vi "RFH-read-general.vi"(7 "file path (dialog if empty)":path, 8 "error in":errorcluster, 11 "sim":bool) -> (0 "error out":errorcluster, 2 "Common Format":T1)   [LabVIEW 2020, in "RFH-Reflection_File_Handler.lvlib"]
doc: "Reads a measurement or simulation file (dialog if the path is empty) into a Common Format cluster; sim marks a simulation file."
uses:
  RFH-Reflection_File_Handler.lvlib
  RFH-common_data_format.ctl
  RFH-libreVNA_data_format.ctl
  <vilib>/Analysis/NI_AALPro.lvlib
panel:
  out "size(s)":i32
  out "real 2":dbl[](graph)
  out "imag 2":dbl[](graph)
  out "mag":dbl[](graph)
  out "phase":dbl[](graph)
  out "imag":dbl[](graph)
  out "real":dbl[](graph)
  out "freq":dbl[](graph)
  out "Array 2":string[](array[string])
  out "string array 3":string[](array[string])
  out "string array 2":string[][](array[string])
  out "string array":string[](array[string])
  out "after substring":string
  out "text":string
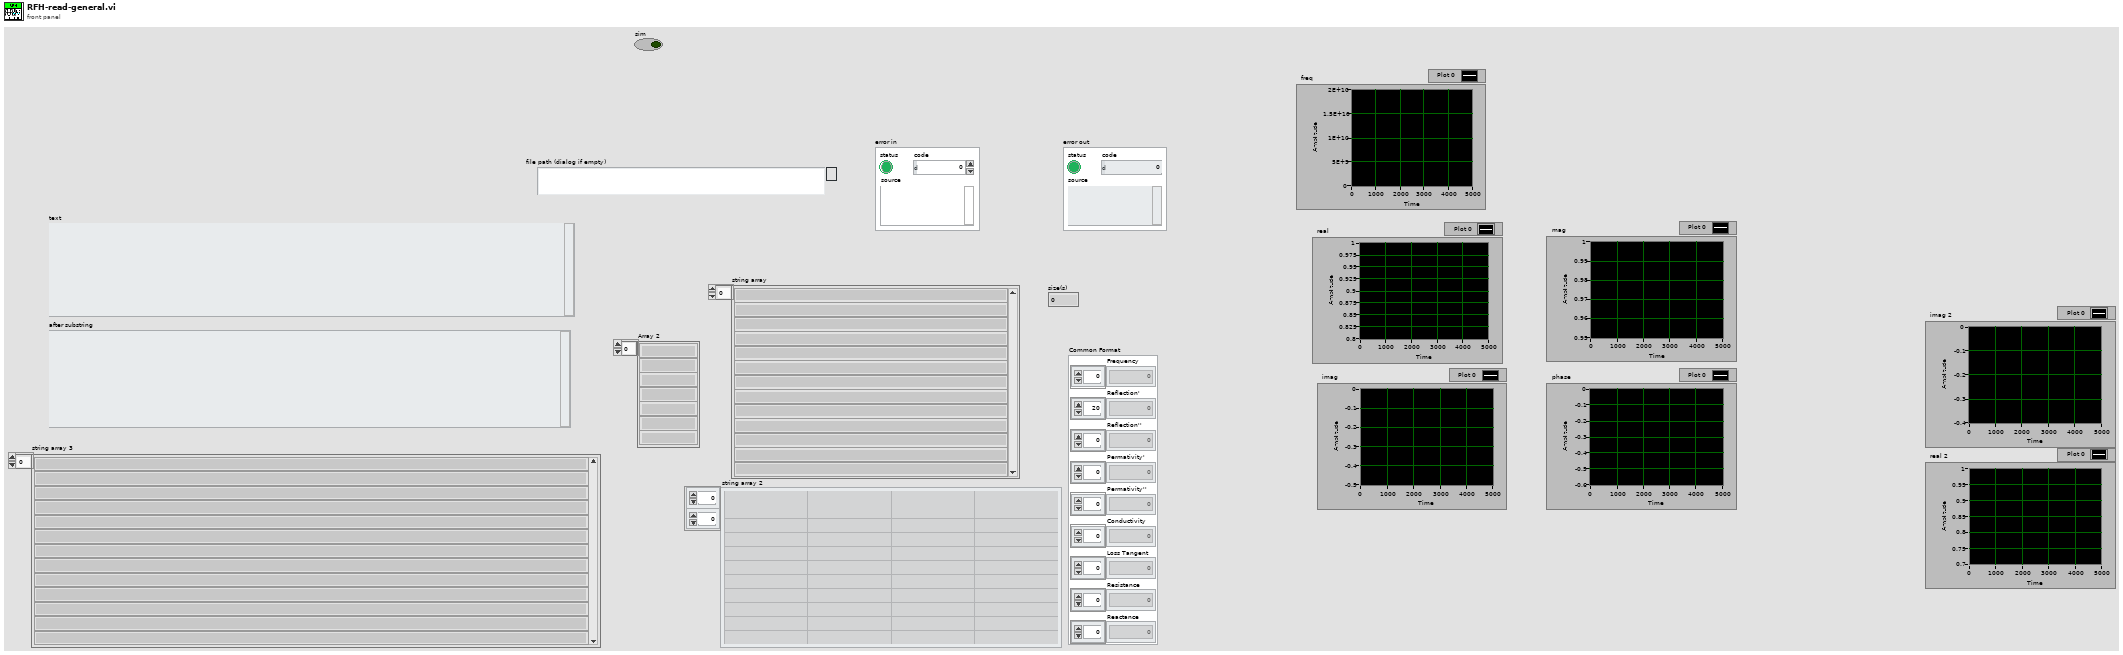
[diagram p1: front panel]
types:
  T1 = typedef "RFH-Reflection_File_Handler.lvlib/RFH-common_data_format.ctl" = cluster{"Frequency":dbl[], "Reflection'":dbl[], "Reflection''":dbl[], "Permativity'":dbl[], "Permativity''":dbl[], "Conductivity":dbl[], "Loss Tangent":dbl[], "Resistance":dbl[], "Reactance":dbl[]}
  T2 = typedef "RFH-Reflection_File_Handler.lvlib/RFH-libreVNA_data_format.ctl" = cluster{"Frequency":dbl[], "S11_Real":dbl[], "S11_Imag":dbl[], "S21_Real":dbl[], "S21_Imag":dbl[], "S12_Real":dbl[], "S12_Imag":dbl[], "S22_Real":dbl[], "S22_Imag":dbl[]}
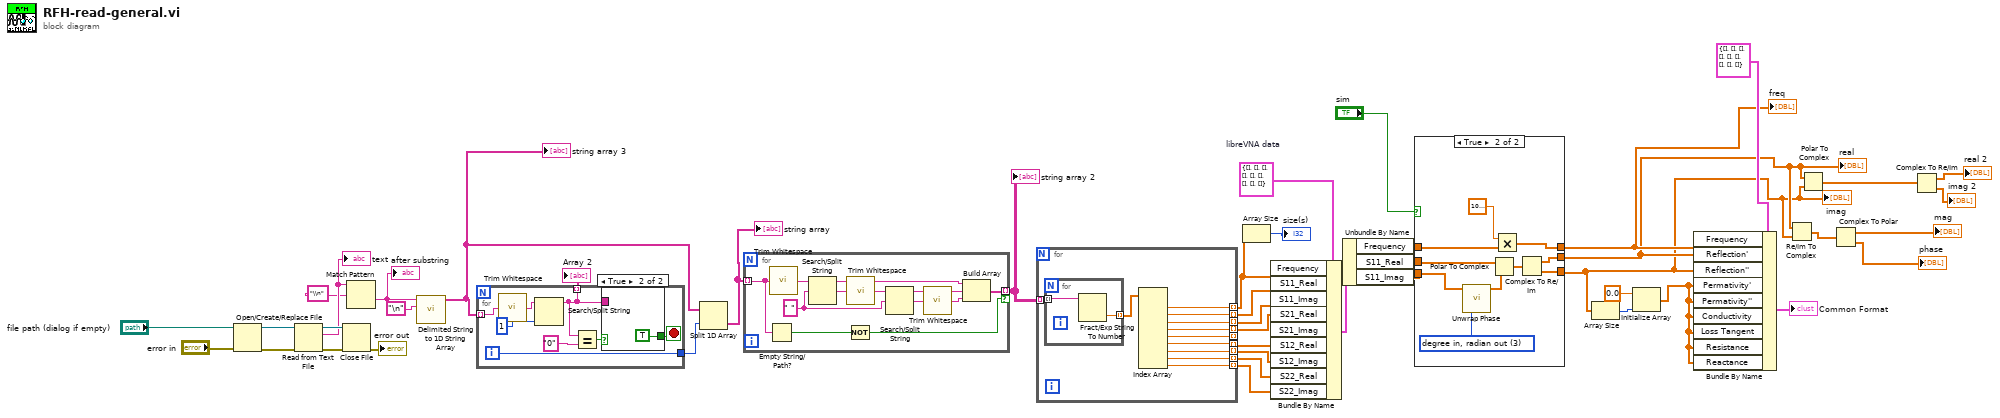
[diagram p0: block diagram]
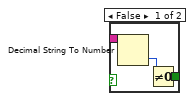
[diagram p3: hidden frame]
diagram:
  w29 = T2 {"Frequency"=[], "S11_Real"=[], "S11_Imag"=[], "S21_Real"=[], "S21_Imag"=[], "S12_Real"=[], "S12_Imag"=[], "S22_Real"=[], "S22_Imag"=[]}  # libreVNA data
  n1 = Open/Create/Replace File(file path (use dialog)="file path (dialog if empty)", error in="error in") -> (refnum out=w46:refnum<file>, error out=w43:errorcluster)  [unwired: 4 in, 1 out]
  n2 = Read from Text File(file (use dialog)=w46, error in=w43) -> (refnum out=w45:refnum<file>, text=w41:string, error out=w44:errorcluster)  [unwired: 2 in, 1 out]
  "text" <- w41
  n3 = Close File(refnum=w45, error in=w44) -> (error out=→"error out":errorcluster)  [unwired: 1 out]
  n4 = Match Pattern(string=w41, regular expression="\\n" ("search string/char (-)")) -> (after substring=w38:string)  [unwired: 1 in, 3 out]
  "after substring" <- w38
  n5 = call <vilib>:"Delimited String to 1D String Array.vi"("delimiter"="\n", "delimited string"=w38) -> ("string array"=w20:string[])  [unwired: 9 in]
  "string array 3" <- w20
  n6 = for {
    tunnel: w20 -> [w52] mode=indexing
    tunnel: [w54] -> w18
    tunnel: [w49] -> w17 mode=indexing
    i -> [w54]
    stop <- w50 stop-if-true
    n7 = call <vilib>:"Trim Whitespace.vi"("string"=w52) -> ("trimmed string"=w51:string)  [unwired: 1 in]
    n8 = Search/Split String(string=w51, offset (0)=1) -> (substring before match=w49:string)  [unwired: 1 in, 2 out]
    n9 = Equal?(x=w49, y="0") -> (x = y?=w47:bool)
    n10 = case shown="True" w47 {
      tunnel: [w56 TRUE] -> w50
      tunnel: w49 -> [w55 _]
      frame False {
        n11 = Decimal String To Number(string=w55) -> (number=w57:i32)  [unwired: 2 in, 1 out]
        n12 = Not Equal To 0?(x=w57) -> (x != 0?=w56:bool)
      }
      frame True {
      }
    }
  }
  "Array 2" <- w17
  n13 = Split 1D Array(array=w20, index=w18) -> (second subarray=w19:string[])  [unwired: 1 out]
  "string array" <- w19
  n14 = for {
    tunnel: w19 -> [w69] mode=indexing
    tunnel: [w59] -> w13 mode=indexing if=w68
    w64 = " " ("search string/char (-)")
    n15 = Empty String/Path?(string/path=w69) -> (empty?=w70:bool)
    n16 = call <vilib>:"Trim Whitespace.vi"("string"=w69) -> ("trimmed string"=w63:string)  [unwired: 1 in]
    n17 = Search/Split String(string=w63, search string/char (-)=w64) -> (substring before match=w62:string, match + rest of string=w66:string)  [unwired: 1 in, 1 out]
    n18 = Not(x=w70) -> (.not. x?=w68:bool)
    n19 = call <vilib>:"Trim Whitespace.vi"("string"=w66) -> ("trimmed string"=w67:string)  [unwired: 1 in]
    n20 = Search/Split String(string=w67, search string/char (-)=w64) -> (substring before match=w61:string, match + rest of string=w65:string)  [unwired: 1 in, 1 out]
    n21 = call <vilib>:"Trim Whitespace.vi"("string"=w65) -> ("trimmed string"=w60:string)  [unwired: 1 in]
    n22 = Build Array(w62, w61, w60) -> (w59:string[])
  }
  "string array 2" <- w13
  n23 = for {
    tunnel: w13 -> [w81] mode=indexing
    tunnel: [w79] -> w9 mode=indexing
    tunnel: [w78] -> w37 mode=indexing
    tunnel: [w77] -> w36 mode=indexing
    tunnel: [w76] -> w35 mode=indexing
    tunnel: [w75] -> w34 mode=indexing
    tunnel: [w74] -> w33 mode=indexing
    tunnel: [w73] -> w32 mode=indexing
    tunnel: [w72] -> w31 mode=indexing
    tunnel: [w71] -> w30 mode=indexing
    n24 = for {
      tunnel: w81 -> [w83] mode=indexing
      tunnel: [w82] -> w80 mode=indexing
      n25 = Fract/Exp String To Number(string=w83) -> (number=w82:dbl)  [unwired: 3 in, 1 out]
    }
    n26 = Index Array(array=w80) -> (element #1=w79:dbl, element #2=w78:dbl, element #3=w77:dbl, element #4=w76:dbl, element #5=w75:dbl, element #6=w74:dbl, element #7=w73:dbl, element #8=w72:dbl, element #9=w71:dbl)  [unwired: 9 in]
  }
  n27 = Array Size(array=w9) -> (size(s)=→"size(s)":i32)
  n28 = Bundle By Name(cluster=w29, "Frequency"=w9, "S11_Real"=w37, "S11_Imag"=w36, "S21_Real"=w35, "S21_Imag"=w34, "S12_Real"=w33, "S12_Imag"=w32, "S22_Real"=w31, "S22_Imag"=w30) -> (w24:T2)
  n29 = Unbundle By Name(w24) -> ("Frequency"=w7:dbl[], "S11_Real"=w6:dbl[], "S11_Imag"=w5:dbl[])
  n30 = case shown="True" "sim" {
    tunnel: w7 -> [w86 w96]
    tunnel: w6 -> [w85 w93]
    tunnel: w5 -> [w84 w89]
    tunnel: [w86 w95] -> w4
    tunnel: [w85 w91] -> w3
    tunnel: [w84 w90] -> w2
    frame False {
    }
    frame True {
      w88 = 3 items=["radian in, radian out", "radian in, degree out", "degree in, degree out", "degree in, radian out"] ("phase unit")
      n31 = call <vilib>:"Unwrap Phase.vi"("phase unit"=w88, "Phase"=w89) -> ("Unwrapped Phase"=w87:dbl[])  [unwired: 8 in, 1 out]
      n32 = Polar To Complex(1:w87, 2:w93) -> (0:w92:cdb[])
      n33 = Multiply(x=1000000000.0 ("element"), y=w96) -> (x*y=w95:dbl[])
      n34 = Complex To Re/Im(x + iy=w92) -> (x=w91:dbl[], y=w90:dbl[])
    }
  }
  "freq" <- w4
  "real" <- w3
  "imag" <- w2
  n35 = Array Size(array=w2) -> (size(s)=w23:i32)
  n36 = Initialize Array(0.0 ("element"), w23) -> (w21:dbl[])
  n37 = Bundle By Name(cluster=T1 {"Frequency"=[], "Reflection'"=[], "Reflection''"=[], "Permativity'"=[], "Permativity''"=[], "Conductivity"=[], "Loss Tangent"=[], "Resistance"=[], "Reactance"=[]} ("Common Format"), "Frequency"=w4, "Reflection'"=w3, "Reflection''"=w2, "Permativity'"=w21, "Permativity''"=w21, "Conductivity"=w21, "Loss Tangent"=w21, "Resistance"=w21, "Reactance"=w21) -> (→"Common Format":T1)
  n38 = Re/Im To Complex(1:w2, 2:w3) -> (0:w16:cdb[])
  n39 = Polar To Complex(1:w2, 2:w3) -> (0:w12:cdb[])
  n40 = Complex To Polar(r * e^(i*theta)=w16) -> (r=→"mag":dbl[], theta=→"phase":dbl[])
  n41 = Complex To Re/Im(x + iy=w12) -> (x=→"real 2":dbl[], y=→"imag 2":dbl[])
